vi "scale analog waveforms.vi"(1 "Scaling parameters":cluster{"Offset":dbl, "Amplitude":dbl}[](array[cluster]), 2 "Analog Waveforms":dbl[][](array[numeric])) -> (0 "Analog Waveforms 2":dbl[][](array[numeric]))   [LabVIEW 2020, in "Scan Generators.lvlib"]
uses:
  Scan Generators.lvlib
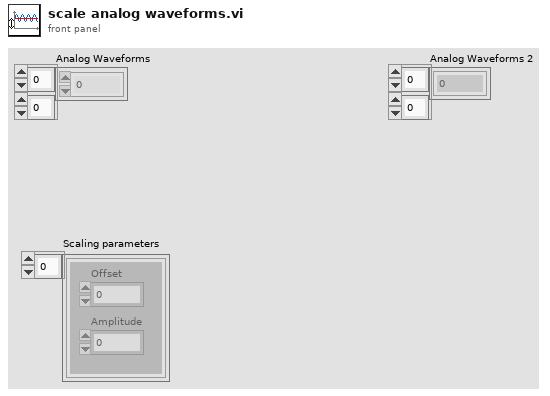
[diagram p1: front panel]
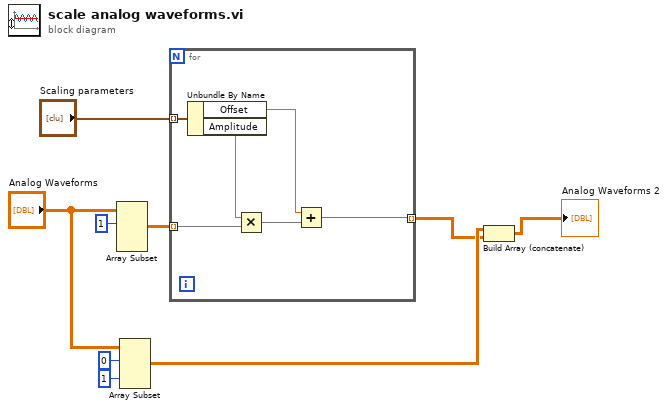
[diagram p0: block diagram]
diagram:
  n1 = Array Subset(array="Analog Waveforms", index (row)=1 ("index")) -> (w7:dbl[][])  [unwired: 3 in]
  n2 = Array Subset(array="Analog Waveforms", index (row)=0 ("index"), length (row)=1 ("length")) -> (w3:dbl[][])  [unwired: 2 in]
  n3 = for {
    tunnel: "Scaling parameters" -> [w15] mode=indexing
    tunnel: w7 -> [w13] mode=indexing
    tunnel: [w10] -> w2 mode=indexing
    n4 = Unbundle By Name(w15) -> ("Offset"=w11:dbl, "Amplitude"=w14:dbl)
    n5 = Multiply(x=w14, y=w13) -> (x*y=w12:dbl[])
    n6 = Add(x=w11, y=w12) -> (x+y=w10:dbl[])
  }
  n7 = Build Array (concatenate)(w3, w2) -> (→"Analog Waveforms 2":dbl[][])
